vi "Configure.vi"(7 "VolatusAPI":refnum<class "VolatusAPI.lvclass">, 8 "error in (no error)":errorcluster, 10 "Config Element":refnum<class "Config Element.lvclass">, 11 "cRIO Power Status EStop in":refnum<class "cRIO Power Status EStop.lvclass">) -> (0 "error out":errorcluster, 3 "cRIO Power Status EStop out":refnum<class "cRIO Power Status EStop.lvclass">)   [LabVIEW 2025, in "VolatusControl.lvlib" / "cRIO Power Status EStop.lvclass"]
uses:
  cRIO Power Status EStop.lvclass
  lv-cdm/CDM-Config/Config Element/Config Element.lvclass
  Volatus/VolatusAPI/VolatusAPI.lvclass
  cRIO Power Status EStop.lvclass/cRIO Power Status EStop.ctl
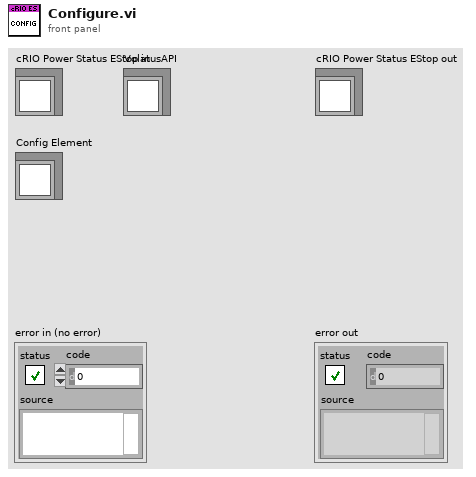
[diagram p1: front panel]
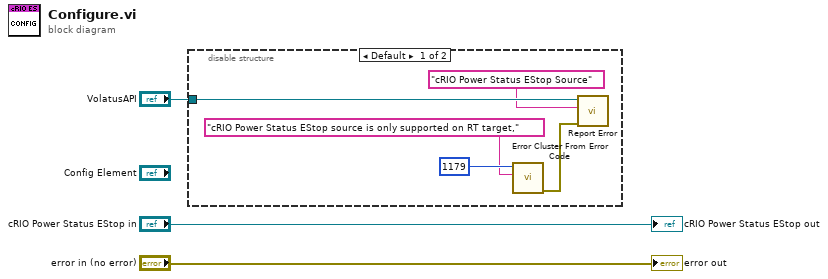
[diagram p0: block diagram]
diagram:
  n1 = disable-structure shown="Default" {
    disable-tunnel: "VolatusAPI" -> [w5 _]
    frame condition #0 (active) {
      n2 = call <vilib>:"Error Cluster From Error Code.vi"("error message (\"\")"="cRIO Power Status EStop source is only supported on RT target," ("error message (\"\")"), "error code (0)"=1179) -> ("error out"=w6:errorcluster)  [unwired: 7 in]
      n3 = call "Report Error.vi"("error in (no error)"=w6, "Context"="cRIO Power Status EStop Source", "VolatusAPI in"=w5) -> ()  [unwired: 7 in, 2 out]
    }
    frame condition #1 {
    }
  }
  "error out" <- "error in (no error)"
  "cRIO Power Status EStop out" <- "cRIO Power Status EStop in"
